vi "cRIO channels Input.vi"() -> ()   [LabVIEW 2025]
panel:
  out "Pressure and Flow meter 2":T1
  out "Temperature\n(C)":T2 {"UUT Discharge temp" format="%0.2f"; "UUT Suction temp" format="%0.2f"; "UUT Liquid temp" format="%0.2f"}
  out "Water Condensed Rate ID":dbl
  out "Diffirential pressure & WFR and Wieght data":T3
  out "RTD Data ID & OD":T4
  in  "Indood TC data":T5
  in  "Outdoor TC data":T6
  # "Discahrge"
  # "Suction"
  # "Liquid"
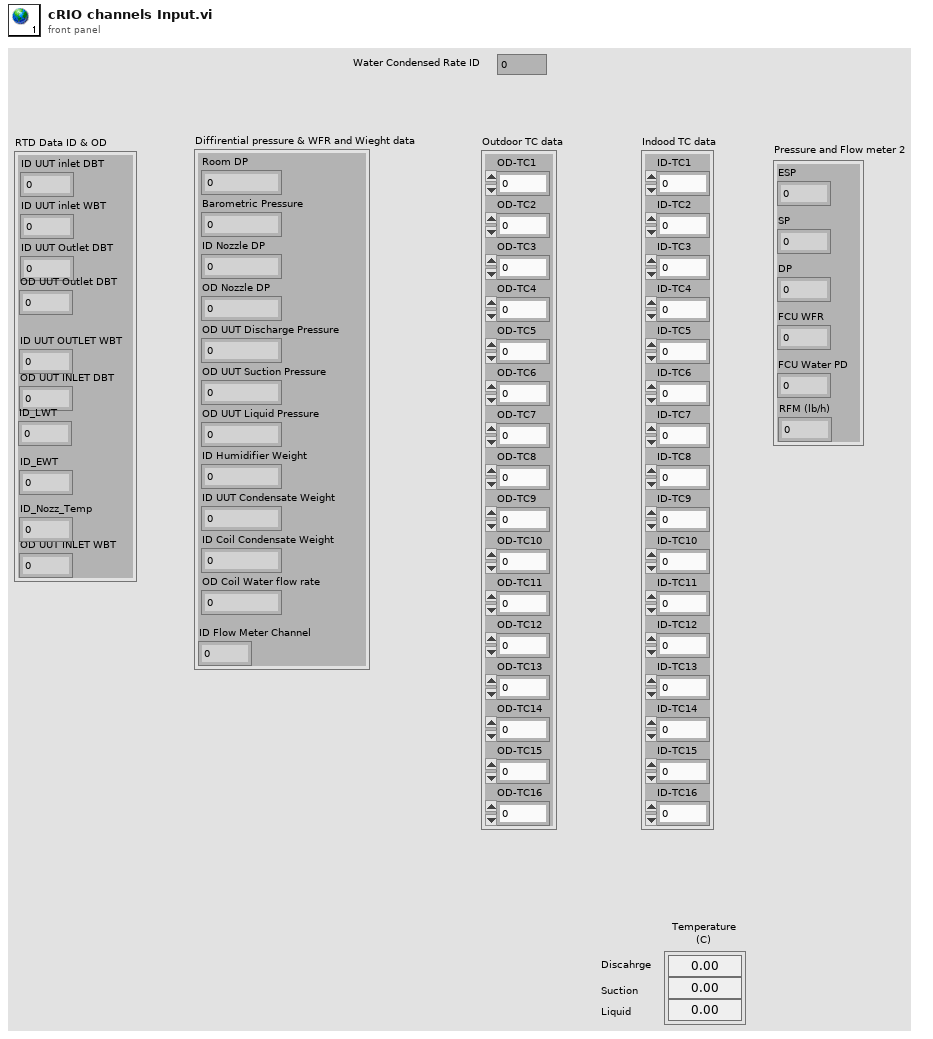
[diagram p1: front panel]
types:
  T1 = cluster{"ESP":dbl, "SP":dbl, "DP":dbl, "FCU WFR":dbl, "FCU Water PD":dbl, "RFM (lb/h)":dbl}
  T2 = cluster{"UUT Liquid temp":dbl, "UUT Suction temp":dbl, "UUT Discharge temp":dbl}
  T3 = cluster{"Room DP":dbl, "Barometric Pressure":dbl, "ID Nozzle DP":dbl, "OD Nozzle DP":dbl, "OD UUT Discharge Pressure":dbl, "OD UUT Suction Pressure":dbl, "OD UUT Liquid Pressure":dbl, "ID Humidifier Weight ":dbl, "ID UUT Condensate Weight":dbl, "ID Coil Condensate Weight":dbl, "OD Coil Water flow rate":dbl, "ID Flow Meter Channel":dbl}
  T4 = cluster{"ID UUT inlet DBT":dbl, "ID UUT inlet WBT":dbl, "ID UUT Outlet DBT":dbl, "OD UUT Outlet DBT":dbl, "ID UUT OUTLET WBT":dbl, "OD UUT INLET DBT":dbl, "OD UUT INLET WBT":dbl, "ID_EWT":dbl, "ID_LWT":dbl, "ID_Nozz_Temp":dbl}
  T5 = cluster{"ID-TC1":dbl, "ID-TC2":dbl, "ID-TC3":dbl, "ID-TC4":dbl, "ID-TC5":dbl, "ID-TC6":dbl, "ID-TC7":dbl, "ID-TC8":dbl, "ID-TC9":dbl, "ID-TC10":dbl, "ID-TC11":dbl, "ID-TC12":dbl, "ID-TC13":dbl, "ID-TC14":dbl, "ID-TC15":dbl, "ID-TC16":dbl}
  T6 = cluster{"OD-TC1":dbl, "OD-TC2":dbl, "OD-TC3":dbl, "OD-TC4":dbl, "OD-TC5":dbl, "OD-TC6":dbl, "OD-TC7":dbl, "OD-TC8":dbl, "OD-TC9":dbl, "OD-TC10":dbl, "OD-TC11":dbl, "OD-TC12":dbl, "OD-TC13":dbl, "OD-TC14":dbl, "OD-TC15":dbl, "OD-TC16":dbl}
diagram:
